vi "Get All Users.vi"(4 "error in (no error)":errorcluster, 7 "EasyUserManager in":refnum<class "EasyUserManager.lvclass">) -> (0 "error out":errorcluster, 2 "Users":string[](array[string]), 3 "EasyUserManager out":refnum<class "EasyUserManager.lvclass">)   [LabVIEW 2024, in "EasyUserManager.lvclass"]
doc: "Read the <B>LoginNames</B> of all users."
uses:
  EasyUserManager.lvclass
  EasyUserManager.lvclass/EasyUserManager.ctl
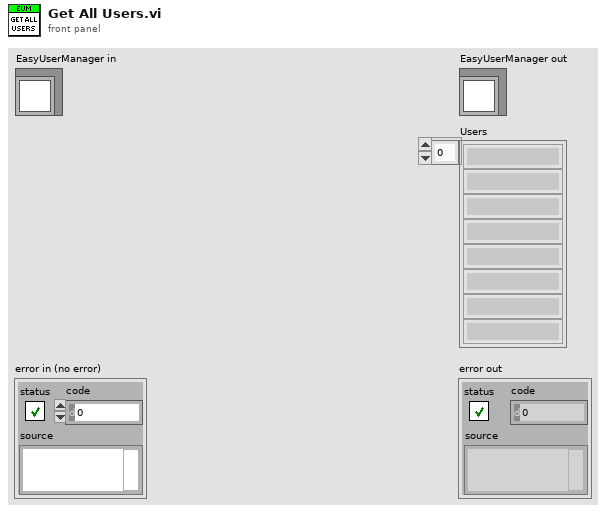
[diagram p1: front panel]
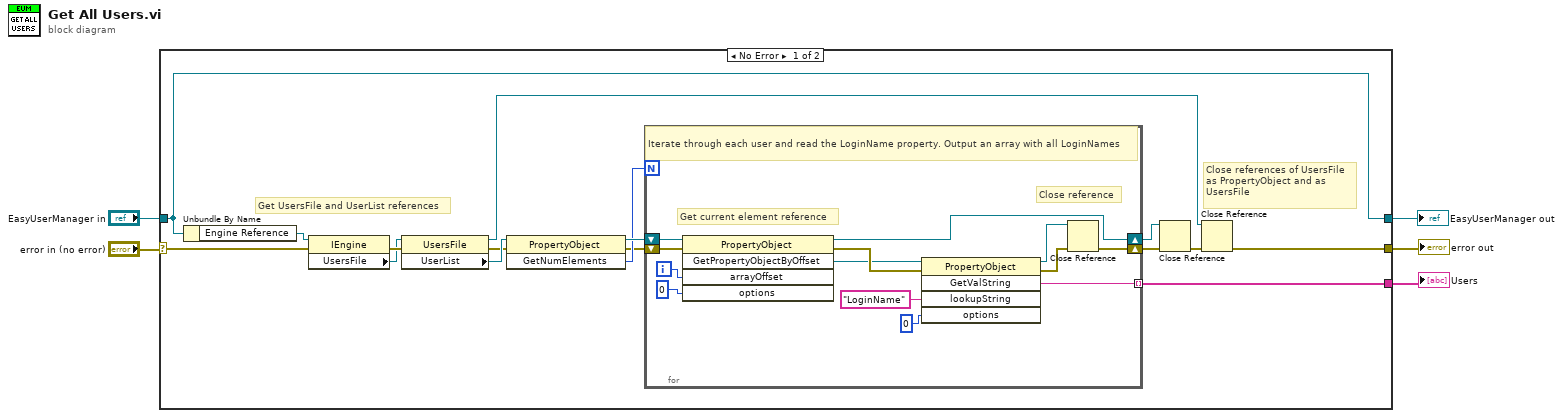
[diagram p0: block diagram]
diagram:
  n1 = case shown="No Error" "error in (no error)" {
    selector: "error in (no error)" -> [w7 w36]
    tunnel: [w10 w36] -> w4
    tunnel: [w9 w35] -> w5
    tunnel: "EasyUserManager in" -> [w9 w35]
    tunnel: [w6 _] -> w1
    frame No Error {
      # "Close references of UsersFile\nas PropertyObject and as\nUsersFile"
      # "Get UsersFile and UserList references"
      n2 = Unbundle By Name(w9) -> ("Engine Reference"=w8:refnum<k7>)
      n3 = property on="Property Node" class="IEngine"(reference=w8, error in=w7) -> (error out=w21:errorcluster, "UsersFile"=w12:refnum<k7>)  [unwired: 1 out]
      n4 = property on="Property Node" class="UsersFile"(reference=w12, error in=w21) -> (reference out=w15:refnum<k7>, error out=w19:errorcluster, "UserList"=w20:refnum<k7>)
      n5 = invoke on="Invoke Node" class="PropertyObject" method="GetNumElements"(reference=w20, error in=w19) -> (reference out=w18:refnum<k7>, error out=w16:errorcluster, "GetNumElements"=w17:i32)  [unwired: 1 in]
      n6 = for {
        N: w17 -> [_]
        shift-right: [w23] -> w11
        shift-left: w16 -> [w22]
        tunnel: [w28] -> w6 mode=indexing
        shift-right: [w26] -> w14
        shift-left: w18 -> [w34]
        i -> [w33]
        # "Get current element reference"
        # "Close reference"
        # "Iterate through each user and read the LoginName property. Output an array with all LoginNames"
        n7 = invoke on="Invoke Node" class="PropertyObject" method="GetPropertyObjectByOffset"(reference=w34, error in=w22, "arrayOffset"=w33, "options"=0) -> (reference out=w26:refnum<k7>, error out=w29:errorcluster, "GetPropertyObjectByOffset"=w27:refnum<k7>)  [unwired: 1 in, 2 out]
        n8 = invoke on="Invoke Node" class="PropertyObject" method="GetValString"(reference=w27, error in=w29, "lookupString"="LoginName", "options"=0) -> (reference out=w25:refnum<k7>, error out=w24:errorcluster, "GetValString"=w28:string)  [unwired: 1 in, 2 out]
        n9 = Close Reference(reference=w25, error in (no error)=w24) -> (error out=w23:errorcluster)
      }
      n10 = Close Reference(reference=w14, error in (no error)=w11) -> (error out=w13:errorcluster)
      n11 = Close Reference(reference=w15, error in (no error)=w13) -> (error out=w10:errorcluster)
    }
    frame Error {
      # "Pass error and do nothing."
    }
  }
  "error out" <- w4
  "EasyUserManager out" <- w5
  "Users" <- w1
